vi "ReadSingleToneProfiles.vi"(7 "模块路径":path, 9 "sn":u16, 10 "错误输入（无错误）":errorcluster, 11 "会话句柄输入":refnum<k35>) -> (2 "错误输出":errorcluster, 3 "会话句柄输出":refnum<k35>, 4 "Single Tone Profiles":T1 {"Single Tone 7"."Phase" step=0.1 format="%.5f"; "Single Tone 7"."Power" min=0.0 max=0.0009998779334127903 step=5e-05 format="%.9f"; "Single Tone 7"."Frequency" min=0.0 max=500000000.0 format="%.7f"; "Single Tone 6"."Phase" step=0.1 format="%.5f"; "Single Tone 6"."Power" min=0.0 max=0.0009998779334127903 step=5e-05 format="%.9f"; "Single Tone 6"."Frequency" min=0.0 max=500000000.0 format="%.7f"; "Single Tone 5"."Phase" step=0.1 format="%.5f"; "Single Tone 5"."Power" min=0.0 max=0.0009998779334127903 step=5e-05 format="%.9f"; "Single Tone 5"."Frequency" min=0.0 max=500000000.0 format="%.7f"; "Single Tone 4"."Phase" step=0.1 format="%.5f"; "Single Tone 4"."Power" min=0.0 max=0.0009998779334127903 step=5e-05 format="%.9f"; "Single Tone 4"."Frequency" min=0.0 max=500000000.0 format="%.7f"; "Single Tone 3"."Phase" step=0.1 format="%.5f"; "Single Tone 3"."Power" min=0.0 max=0.0009998779334127903 step=5e-05 format="%.9f"; "Single Tone 3"."Frequency" min=0.0 max=500000000.0 format="%.7f"; "Single Tone 2"."Phase" step=0.1 format="%.5f"; "Single Tone 2"."Power" min=0.0 max=0.0009998779334127903 step=5e-05 format="%.9f"; "Single Tone 2"."Frequency" min=0.0 max=500000000.0 format="%.7f"; "Single Tone 1"."Phase" step=0.1 format="%.5f"; "Single Tone 1"."Power" min=0.0 max=0.0009998779334127903 step=5e-05 format="%.9f"; "Single Tone 1"."Frequency" min=0.0 max=500000000.0 format="%.7f"; "Single Tone 0"."Phase" step=0.1 format="%.5f"; "Single Tone 0"."Power" min=0.0 max=0.0009998779334127903 step=5e-05 format="%.9f"; "Single Tone 0"."Frequency" min=0.0 max=500000000.0 format="%.7f"}, 5 "Activate":T2(radio))   [LabVIEW 2018]
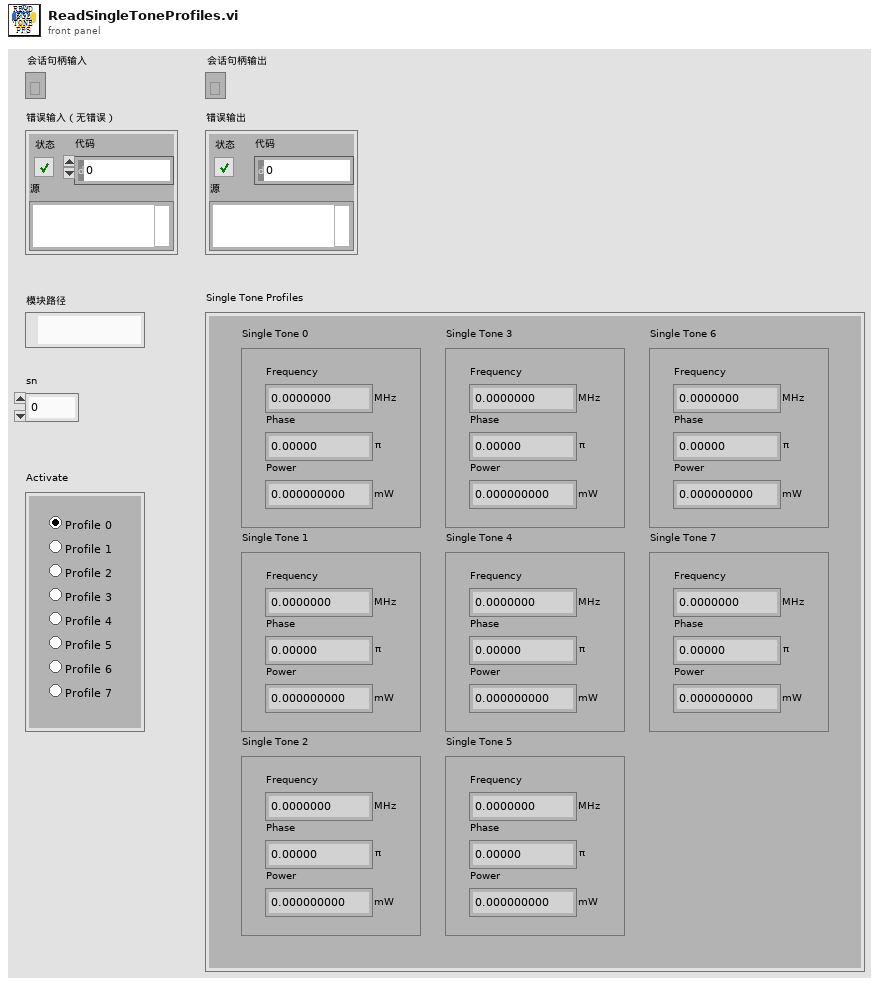
[diagram p1: front panel]
types:
  T1 = cluster{"Single Tone 0":cluster{"Frequency":dbl[unit], "Phase":dbl, "Power":dbl[unit]}, "Single Tone 1":cluster{"Frequency":dbl[unit], "Phase":dbl, "Power":dbl[unit]}, "Single Tone 2":cluster{"Frequency":dbl[unit], "Phase":dbl, "Power":dbl[unit]}, "Single Tone 3":cluster{"Frequency":dbl[unit], "Phase":dbl, "Power":dbl[unit]}, "Single Tone 4":cluster{"Frequency":dbl[unit], "Phase":dbl, "Power":dbl[unit]}, "Single Tone 5":cluster{"Frequency":dbl[unit], "Phase":dbl, "Power":dbl[unit]}, "Single Tone 6":cluster{"Frequency":dbl[unit], "Phase":dbl, "Power":dbl[unit]}, "Single Tone 7":cluster{"Frequency":dbl[unit], "Phase":dbl, "Power":dbl[unit]}}
  T2 = enum32{"单选选项0", "单选选项1", "单选选项2", "单选选项3", "单选选项4", "单选选项5", "单选选项6", "单选选项7"}
  T3 = cluster{"数值":u8, "数组":cluster{"数值":dbl, "数值 2":dbl, "数值 3":dbl}[]}
  T4 = cluster{"[0]":cluster{dbl[unit], "数值 2":dbl, dbl[unit]}, "[1]":cluster{dbl[unit], "数值 2":dbl, dbl[unit]}, "[2]":cluster{dbl[unit], "数值 2":dbl, dbl[unit]}, "[3]":cluster{dbl[unit], "数值 2":dbl, dbl[unit]}, "[4]":cluster{dbl[unit], "数值 2":dbl, dbl[unit]}, "[5]":cluster{dbl[unit], "数值 2":dbl, dbl[unit]}, "[6]":cluster{dbl[unit], "数值 2":dbl, dbl[unit]}, "[7]":cluster{dbl[unit], "数值 2":dbl, dbl[unit]}}
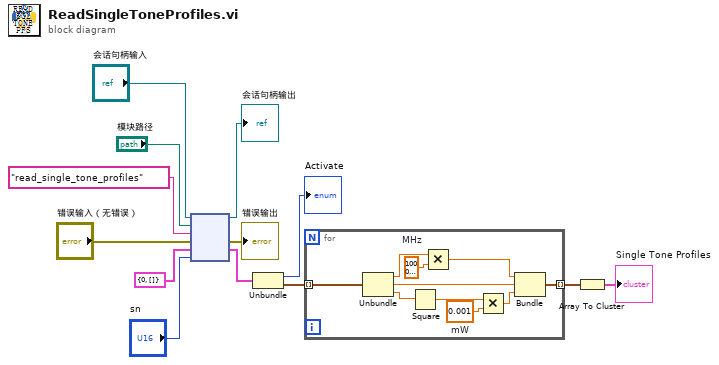
[diagram p0: block diagram]
diagram:
  n1 = node("会话句柄输入", "模块路径", "read_single_tone_profiles", "错误输入（无错误）", T3 {"数值"=0, "数组"=[]} ("簇"), "sn") -> (→"会话句柄输出":refnum<k35>, →"错误输出":errorcluster, w6:T3)  [unwired: 1 in, 2 out]
  n2 = Unbundle(w6) -> ("数值"=→"Activate":u8, "数组"=w4:cluster{"数值":dbl, "数值 2":dbl, "数值 3":dbl}[])
  n3 = for {
    tunnel: w4 -> [w23] mode=indexing
    tunnel: [w18] -> w3 mode=indexing
    w15 = dbl[unit] 0.001  # mW
    w17 = dbl[unit] 1000000.0  # MHz
    n4 = Unbundle(w23) -> ("数值"=w16:dbl, "数值 2"=w20:dbl, "数值 3"=w22:dbl)
    n5 = Square(x=w22) -> (x^2=w14:dbl)
    n6 = Multiply(x=w16, y=w17) -> (x*y=w21:dbl[unit])
    n7 = Multiply(x=w14, y=w15) -> (x*y=w19:dbl[unit])
    n8 = Bundle(w21, "数值 2"=w20, w19) -> (w18:cluster{dbl[unit], "数值 2":dbl, dbl[unit]})  [unwired: 1 in]
  }
  n9 = Array To Cluster(array=w3) -> (cluster=→"Single Tone Profiles":T4)
